vi "enkoder.vi"() -> ()   [LabVIEW 2025]
panel:
  out "Message with CRC":u32 format="%b"
  out "CRC":u32 format="%b"
  out "maska":u32 format="%b"
  in  "Stop":bool
  in  "D":u32 format="%b"
  in  "P":u32 format="%b"
  out "Message":u32 format="%b"
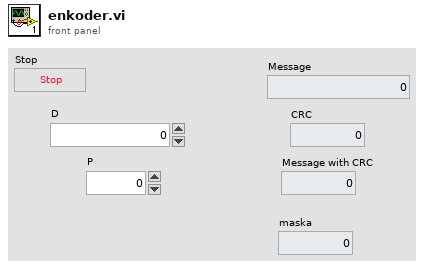
[diagram p1: front panel]
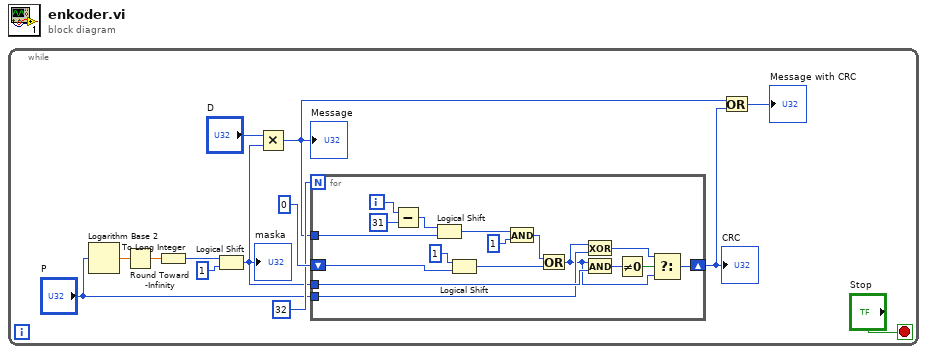
[diagram p0: block diagram]
diagram:
  n1 = while {
    stop <- "Stop" stop-if-true
    n2 = Logarithm Base 2(1:"P") -> (0:w12:dbl)
    n3 = Round Toward -Infinity(1:w12) -> (0:w11:dbl)
    n4 = To Long Integer(number=w11) -> (32bit integer=w9:i32)
    n5 = Logical Shift(y=w9, x=u32 1) -> (x << y=w4:u32)
    "maska" <- w4
    n6 = Multiply(x="D", y=w4) -> (x*y=w3:u32)
    "Message" <- w3
    n7 = for {
      N: 32 -> [_]
      shift-right: [w14] -> w2
      shift-left: u32 0 -> [w24]
      tunnel: w3 -> [w30]
      tunnel: "P" -> [w17]
      tunnel: w4 -> [w20]
      i -> [w29]
      n8 = Subtract(x=w29, y=31) -> (x-y=w27:i32)
      n9 = Logical Shift(y=w27, x=w30) -> (x << y=w26:u32)
      n10 = Logical Shift(y=i16 1, x=w24) -> (x << y=w22:u32)
      n11 = And(x=w26, y=u32 1) -> (x .and. y?=w21:u32)
      n12 = Or(x=w21, y=w22) -> (x .or. y?=w15:u32)
      n13 = Exclusive Or(1:w17, 2:w15) -> (0:w16:u32)
      n14 = And(x=w15, y=w20) -> (x .and. y?=w19:u32)
      n15 = Not Equal To 0?(x=w19) -> (x != 0?=w18:bool)
      n16 = Select(t=w16, s=w18, f=w15) -> (s? t:f=w14:u32)
    }
    "CRC" <- w2
    n17 = Or(x=w3, y=w2) -> (x .or. y?=→"Message with CRC":u32)
  }
